vi "SensorDetectColor.vi"(0 "Color":T1=enum."Blue", 2 "NXT/EV3 IN":T3, 3 "Port":T2 items=["Port 1", "Port 2", "Port 3", "Port 4"]) -> (1 "Out":bool, 4 "NXT/EV3 OUT":T3)   [LabVIEW 2016, in "13.03 Robot.lvrbt"]
uses:
  13.03 Robot.lvrbt
  <vilib>/NXT/Subs/LVHSConnector.ctl
  <vilib>/NXT/LegoClasses/BrickReference/BrickReference.lvclass
  <vilib>/NXT/Block Support/NXT_InputPort.ctl
  <vilib>/NXT/Subs/ColorSensorColors.ctl
  <vilib>/NXT/Dual Mode Library/Sensors/EV3_Color_Color.vi
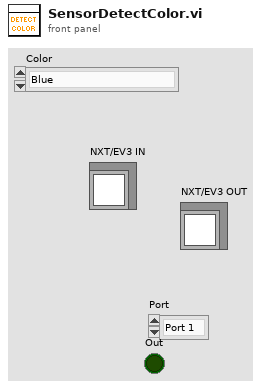
[diagram p1: front panel]
types:
  T1 = typedef "ColorSensorColors.ctl" = enum16{"No Color", "Black", "Blue", "Green", "Yellow", "Red", "White", "Brown"}
  T2 = typedef "NXT_InputPort.ctl" = u32
  T3 = typedef "LVHSConnector.ctl" = refnum<class "BrickReference.lvclass">
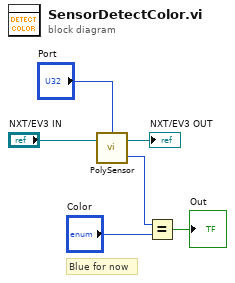
[diagram p0: block diagram]
diagram:
  # "Blue for now"
  n1 = call-poly <vilib>:"PolySensor.vi"("NXT/EV3"="NXT/EV3 IN", "Port (Port 1)"="Port") -> ("Detected Color"=w3:T1, "NXT/EV3"=→"NXT/EV3 OUT":T3)  [unwired: 1 in]
  n2 = Equal?(x=w3, y="Color") -> (x = y?=→"Out":bool)
